vi "Initialize Monitor.vi"(8 "error in (no error)":errorcluster, 10 "Target Ref in":T7 format="%.0x", 11 "Addon Ref in":T7 format="%.0x") -> (0 "error out":errorcluster, 2 "Found?":bool, 3 "Monitor Frame Configurations":T1[](array[typedef]) {"Validation Channels Refs"."Data Reference" format="%.0x"; "CD Results Refs"."Data Reference" format="%.0x"; "Input Channels Refs"."Data Reference" format="%.0x"; "Frame Configuration"."CRC"."Data Type" items=["Signed", "Unsigned", "IEEE Float"]; "Frame Configuration"."Rolling Counter"."Data Type" items=["Signed", "Unsigned", "IEEE Float"]; "Frame Configuration"."Input Channels"."Data Type" items=["Signed", "Unsigned", "IEEE Float"]})   [LabVIEW 2015, in "Protection and Rolling Counter Addon Engine.lvlib"]
uses:
  Protection and Rolling Counter Addon Engine.lvlib
  <vilib>/NI Veristand/Custom Device API/Custom Device Item Ref.ctl
  Types/RT Engine Monitor References.ctl
  Shared/Types/FrameConfiguration.ctl
  Shared/Types/InputChannelConfiguration.ctl
  Shared/Types/Protection Type.ctl
  <vilib>/NI Veristand/Custom Device API/Block Data Reference.ctl
  <vilib>/NI Veristand/Custom Device API/Data Reference.ctl
  <vilib>/NI Veristand/Custom Device Tools/Custom Device Utility Library/Search Direction.ctl
  <vilib>/NI Veristand/Custom Device API/Data Access Type.ctl
  Shared/SubVIs/GUID Lookup.vi
  <vilib>/NI Veristand/Custom Device Tools/Custom Device Utility Library/NI VeriStand - Search for Item by GUID.vi
  <vilib>/NI Veristand/Custom Device Tools/Custom Device Utility Library/NI VeriStand - Search for All Items by GUID.vi
  <vilib>/xnet/xnet.llb/XNET Create Session (Conversion).vi
  <vilib>/NI Veristand/Custom Device Tools/Custom Device Utility Library/Custom Device Utility Library.lvlib
  Shared/Protection and Rolling Counter Addon Shared.lvlib
  <vilib>/NI Veristand/Custom Device API/Custom Device API.lvlib
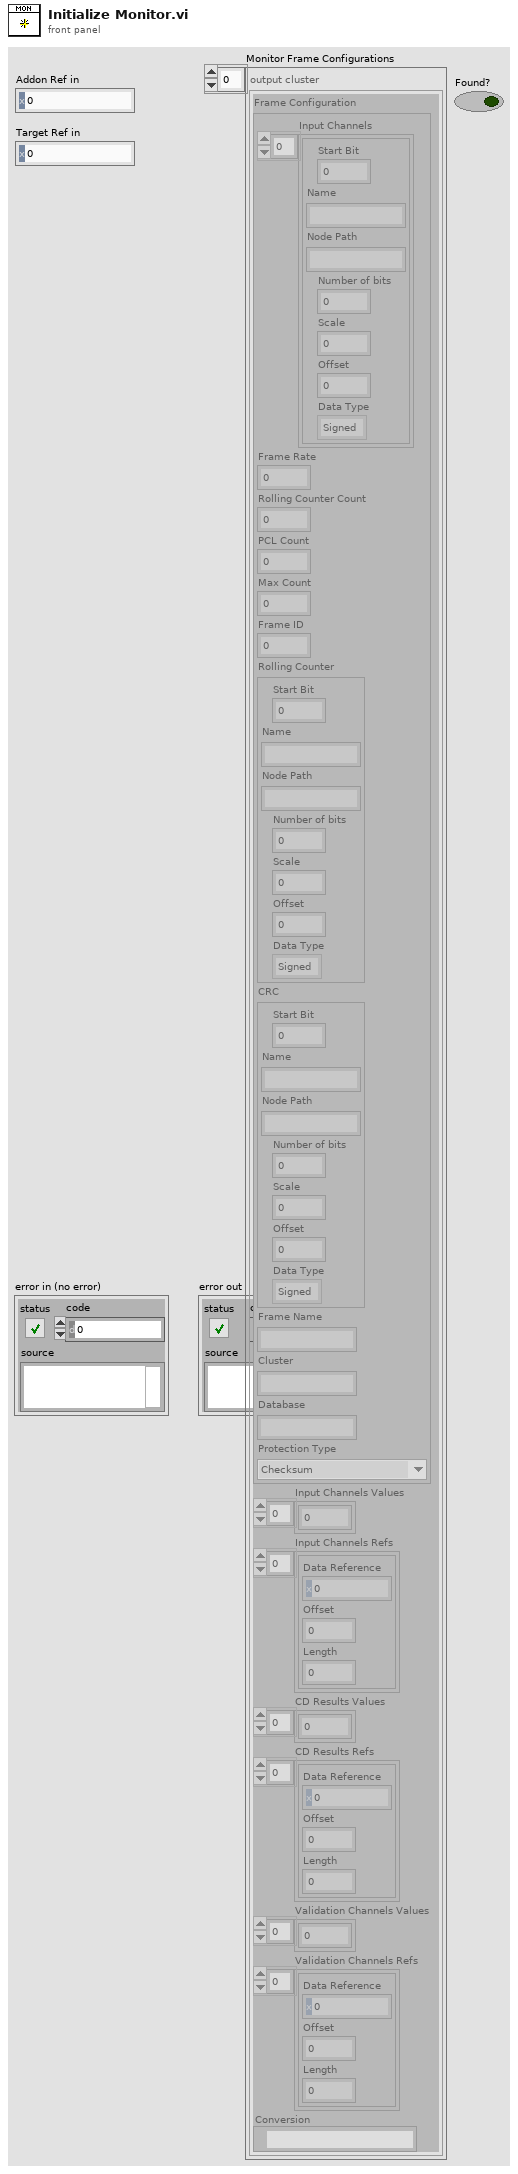
[diagram p1: front panel]
types:
  T1 = typedef "Protection and Rolling Counter Addon Engine.lvlib/RT Engine Monitor References.ctl" = cluster{"Frame Configuration":T2, "Input Channels Values":dbl[], "Input Channels Refs":T5[], "CD Results Values":dbl[], "CD Results Refs":T5[], "Validation Channels Values":dbl[], "Validation Channels Refs":T5[], "Conversion":refnum<k21>}
  T2 = typedef "Protection and Rolling Counter Addon Shared.lvlib/FrameConfiguration.ctl" = cluster{"Input Channels":T3[], "Frame Rate":dbl, "Rolling Counter Count":dbl, "PCL Count":u64, "Max Count":dbl, "Frame ID":u32, "Rolling Counter":T3, "CRC":T3, "Frame Name":string, "Cluster":string, "Database":string, "Protection Type":T4}
  T3 = typedef "Protection and Rolling Counter Addon Shared.lvlib/InputChannelConfiguration.ctl" = cluster{"Start Bit":i32, "Name":string, "Node Path":string, "Number of bits":i32, "Scale":dbl, "Offset":dbl, "Data Type":u32}
  T4 = typedef "Protection and Rolling Counter Addon Shared.lvlib/Protection Type.ctl" = enum16{"Checksum", "CRC", "None (Counter Only)"}
  T5 = typedef "Custom Device API.lvlib/Block Data Reference.ctl" = cluster{"Data Reference":T6, "Offset":u64, "Length":u64}
  T6 = typedef "Custom Device API.lvlib/Data Reference.ctl" = i32
  T7 = typedef "Custom Device API.lvlib/Custom Device Item Ref.ctl" = u64
  T8 = typedef "Custom Device Utility Library.lvlib/Search Direction.ctl" = enum16{"Down", "Up"}
  T9 = typedef "Custom Device API.lvlib/Data Access Type.ctl" = enum16{"Read", "Write"}
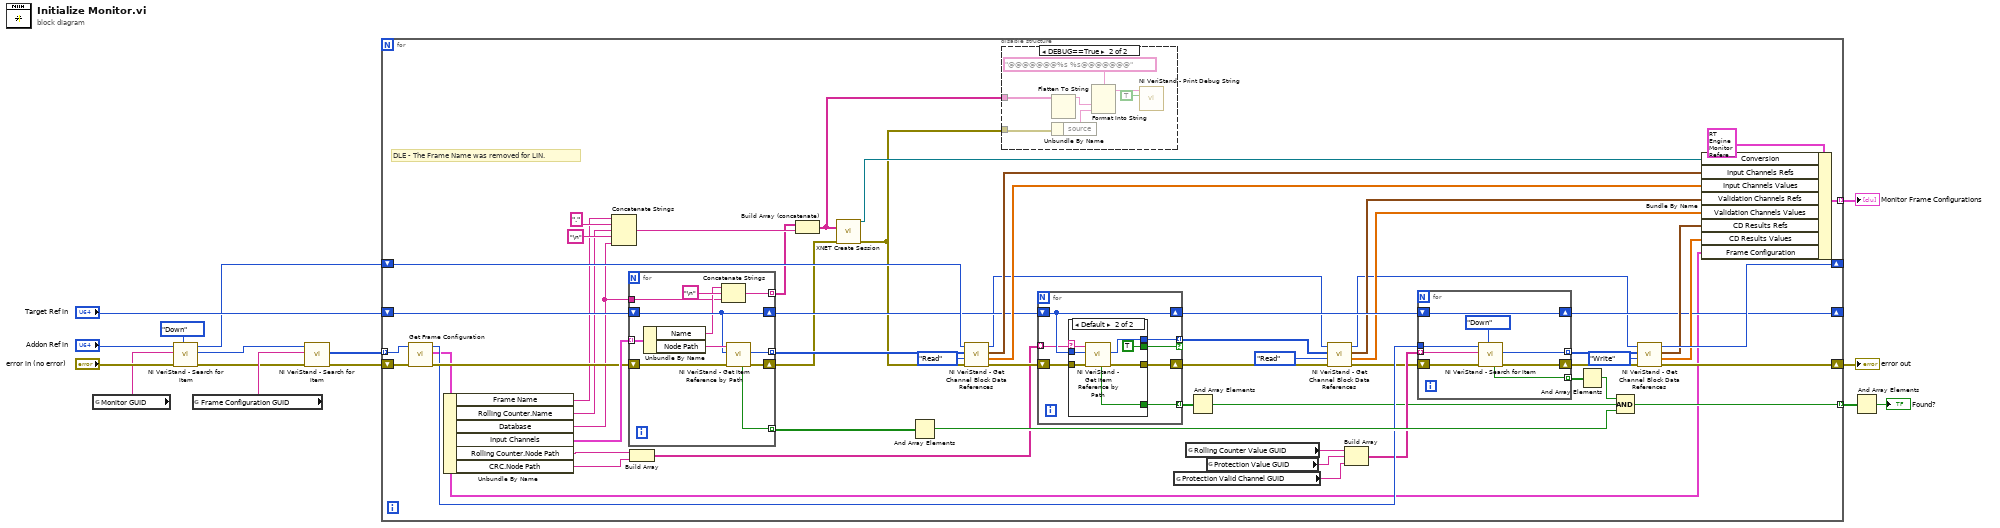
[diagram p0: block diagram]
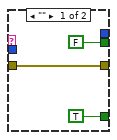
[diagram p3: hidden frame]
diagram:
  n1 = global read "GUID Lookup.vi" "Monitor GUID"() -> (w4:string)
  n2 = call-poly <vilib>:"NI VeriStand - Search for Item.vi"("Direction (Down)"=Search_Direction."Down", "error in"="error in (no error)", "Item GUID"=w4, "Section Ref in"="Addon Ref in") -> ("error out"=w8:errorcluster, "Item Ref"=w6:T7, "Section Ref out"=w5:T7)  [unwired: 4 in, 1 out]
  n3 = global read "GUID Lookup.vi" "Frame Configuration GUID"() -> (w10:string)
  n4 = call-poly <vilib>:"NI VeriStand - Search for Item.vi"("error in"=w8, "Item GUID"=w10, "Section Ref in"=w6) -> ("error out"=w11:errorcluster, "Item Refs"=w12:T7[])  [unwired: 5 in, 2 out]
  n5 = for {
    shift-right: [w54] -> w14
    shift-left: w11 -> [w73]
    tunnel: w12 -> [w72] mode=indexing
    shift-right: [w64] -> _
    shift-left: w5 -> [w51]
    tunnel: [w57] -> w1 mode=indexing
    tunnel: [w59] -> w13 mode=indexing
    shift-right: [w46] -> _
    shift-left: "Target Ref in" -> [w53]
    # "DLE - The Frame Name was removed for LIN."
    n6 = call "Get Frame Configuration.vi"("error in"=w73, "Parent Ref"=w72) -> ("error out"=w52:errorcluster, "Selected Channels"=w21:T2, "Parent Ref Out"=w50:T7)  [unwired: 7 in]
    n7 = Unbundle By Name(w21) -> ("Frame Name"=w16:string, "Rolling Counter.Name"=w25:string, "Database"=w23:string, "Input Channels"=w71:T3[], "Rolling Counter.Node Path"=w37:string, "CRC.Node Path"=w36:string)
    n8 = Concatenate Strings(w16, "." ("string"), w25, "\n" ("string"), w23) -> (w26:string)
    n9 = for {
      tunnel: w71 -> [w116] mode=indexing
      shift-right: [w112] -> w24
      shift-left: w52 -> [w115]
      shift-right: [w110] -> w39
      shift-left: w53 -> [w110]
      tunnel: [w114] -> w67 mode=indexing
      tunnel: [w113] -> w70 mode=indexing
      tunnel: w23 -> [w107]
      tunnel: [w106] -> w22 mode=indexing
      n10 = Unbundle By Name(w116) -> ("Name"=w108:string, "Node Path"=w111:string)
      n11 = Concatenate Strings(w108, "\n" ("string"), w107) -> (w106:string)
      n12 = call <vilib>:"NI VeriStand - Get Item Reference by Path.vi"("error in (no error)"=w115, "Root Ref"=w110, "Item Path in"=w111) -> ("error out"=w112:errorcluster, "Item Ref"=w114:T7, "Found"=w113:bool)  [unwired: 5 in, 1 out]
    }
    n13 = Build Array(w37, w36) -> (w35:string[])
    n14 = Build Array (concatenate)(w22, w26) -> (w19:string[])
    n15 = call-poly <vilib>:"XNET Create Session.vi"("signal list"=w19, "error in (no error)"=w24) -> ("session out"=w20:refnum<k21>, "error out"=w18:errorcluster)  [unwired: 12 out]
    n16 = And Array Elements(Boolean array=w70) -> (logical AND=w69:bool)
    n17 = call <vilib>:"NI VeriStand - Get Channel Block Data References.vi"("error in (no error)"=w18, "Access"=Data_Access_Type."Read", "Channel Refs"=w67, "Device Ref in"=w51) -> ("error out"=w41:errorcluster, "Values Array"=w65:dbl[], "Block Data Refs"=w66:T5[], "Device Ref out"=w30:T7)  [unwired: 4 in]
    n18 = disable-structure shown="DEBUG==True" {
      disable-tunnel: w18 -> [_ w79]
      disable-tunnel: w19 -> [_ w77]
      frame condition #0 (active) {
      }
      frame condition #1 {
        n19 = Flatten To String(anything=w77) -> (data string=w76:string)  [unwired: 3 in, 2 out]
        n20 = Unbundle By Name(w79) -> ("source"=w75:string)
        n21 = Format Into String(format string="@@@@@@@%s %s@@@@@@@", w76, w75) -> (resulting string=w74:string)  [unwired: 2 in, 1 out]
        n22 = call <vilib>:"NI VeriStand - Print Debug String.vi"("Add to log file? (T)"=TRUE, "Message"=w74) -> ()  [unwired: 9 in, 1 out]
      }
    }
    n23 = for {
      shift-right: [w84] -> w44
      shift-left: w41 -> [w87]
      shift-right: [w83] -> w38
      shift-left: w39 -> [w83]
      tunnel: [w86] -> w28 mode=indexing if=w81
      tunnel: [w85] -> w42 mode=indexing
      tunnel: w35 -> [w82] mode=indexing
      n24 = case shown="Default" w82 {
        selector: w82 -> [_ w92]
        tunnel: w87 -> [w90 w97]
        tunnel: [_ w96] -> w86
        tunnel: [TRUE ("Found") w95] -> w85
        tunnel: [w90 w94] -> w84
        tunnel: w83 -> [_ w93]
        tunnel: [FALSE TRUE] -> w81
        frame "" {
        }
        frame Default {
          n25 = call <vilib>:"NI VeriStand - Get Item Reference by Path.vi"("error in (no error)"=w97, "Root Ref"=w93, "Item Path in"=w92) -> ("error out"=w94:errorcluster, "Item Ref"=w96:T7, "Found"=w95:bool)  [unwired: 5 in, 1 out]
        }
      }
    }
    n26 = global read "GUID Lookup.vi" "Protection Valid Channel GUID"() -> (w45:string)
    n27 = global read "GUID Lookup.vi" "Rolling Counter Value GUID"() -> (w49:string)
    n28 = And Array Elements(Boolean array=w42) -> (logical AND=w31:bool)
    n29 = global read "GUID Lookup.vi" "Protection Value GUID"() -> (w48:string)
    n30 = call <vilib>:"NI VeriStand - Get Channel Block Data References.vi"("error in (no error)"=w44, "Access"=Data_Access_Type."Read", "Channel Refs"=w28, "Device Ref in"=w30) -> ("error out"=w40:errorcluster, "Values Array"=w32:dbl[], "Block Data Refs"=w33:T5[], "Device Ref out"=w29:T7)  [unwired: 4 in]
    n31 = Build Array(w49, w48, w45) -> (w47:string[])
    n32 = for {
      shift-right: [w103] -> w55
      shift-left: w40 -> [w104]
      shift-right: [w105] -> w46
      shift-left: w38 -> [w105]
      tunnel: [w101] -> w60 mode=indexing
      tunnel: [w102] -> w58 mode=indexing
      tunnel: w50 -> [w100]
      tunnel: w47 -> [w99] mode=indexing
      n33 = call-poly <vilib>:"NI VeriStand - Search for Item.vi"("Direction (Down)"=Search_Direction."Down", "error in"=w104, "Item GUID"=w99, "Section Ref in"=w100) -> ("error out"=w103:errorcluster, "Item Ref"=w101:T7, "Found"=w102:bool)  [unwired: 4 in, 1 out]
    }
    n34 = And Array Elements(Boolean array=w58) -> (logical AND=w56:bool)
    n35 = Compound Arithmetic op=AND(w56, w31, w69) -> (w57:bool)
    n36 = call <vilib>:"NI VeriStand - Get Channel Block Data References.vi"("error in (no error)"=w55, "Access"=Data_Access_Type."Write", "Channel Refs"=w60, "Device Ref in"=w29) -> ("error out"=w54:errorcluster, "Values Array"=w61:dbl[], "Block Data Refs"=w62:T5[], "Device Ref out"=w64:T7)  [unwired: 4 in]
    n37 = Bundle By Name(cluster=T1 {"Frame Configuration"={"Input Channels"=[], "Frame Rate"=0.0, "Rolling Counter Count"=0.0, "PCL Count"=0, "Max Count"=0.0, "Frame ID"=0, "Rolling Counter"={"Start Bit"=0, "Name"="", "Node Path"="", "Number of bits"=0, "Scale"=0.0, "Offset"=0.0, "Data Type"=0}, "CRC"={"Start Bit"=0, "Name"="", "Node Path"="", "Number of bits"=0, "Scale"=0.0, "Offset"=0.0, "Data Type"=0}, "Frame Name"="", "Cluster"="", "Database"="", "Protection Type"=enum."Checksum"}, "Input Channels Values"=[], "Input Channels Refs"=[], "CD Results Values"=[], "CD Results Refs"=[], "Validation Channels Values"=[], "Validation Channels Refs"=[], "Conversion"=""} ("output cluster"), "Conversion"=w20, "Input Channels Refs"=w66, "Input Channels Values"=w65, "Validation Channels Refs"=w33, "Validation Channels Values"=w32, "CD Results Refs"=w62, "CD Results Values"=w61, "Frame Configuration"=w21) -> (w59:T1)
  }
  "error out" <- w14
  "Monitor Frame Configurations" <- w13
  n38 = And Array Elements(Boolean array=w1) -> (logical AND=→"Found?":bool)
